vi "Sreen.vi"(1 "IP":string, 2 "Voltage 2":u8, 3 "Voltage 1":u8, 4 "Battery":u8) -> ()   [LabVIEW 2024]
panel:
  out "Port":dbl
  in  "Send":bool
  # "OED Screen Control"
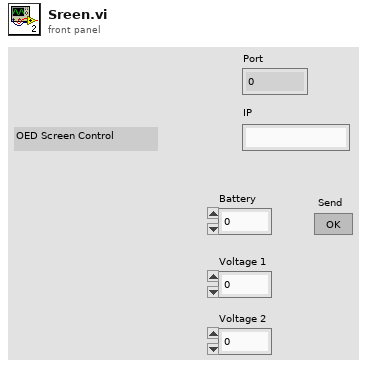
[diagram p1: front panel]
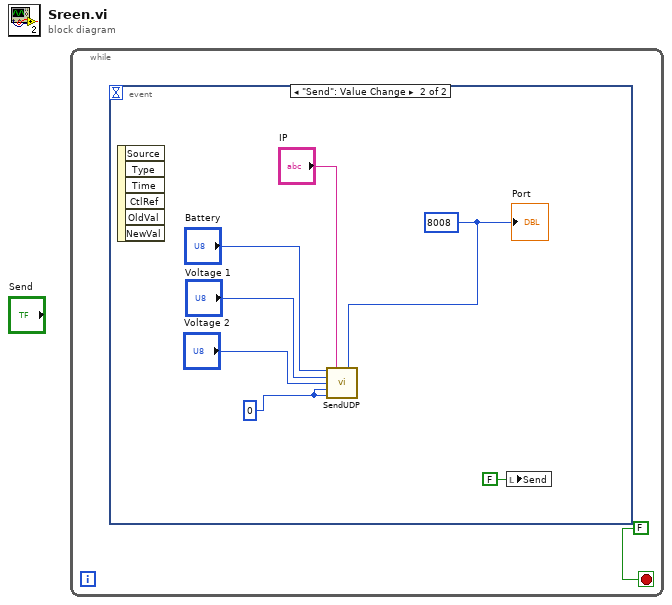
[diagram p0: block diagram]
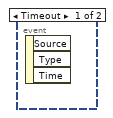
[diagram p2: hidden frame]
diagram:
  n1 = while {
    stop <- FALSE stop-if-true
    n2 = event shown="[1] \"Send\": Value Change" {
      selector: _ -> [_ _]
      dyn-events: _ -> [_ _]
      timeout: _ -> [_ _]
      event Timeout {
        n3 = event-data() -> ()  [unwired: 1 in, 3 out]
      }
      event "Send": Value Change {
        w2 = 0
        w7 = 8008
        n4 = event-data() -> ()  [unwired: 1 in, 6 out]
        n5 = call "SendUDP.vi"("Arg3"="Battery", "IP"="IP", "Port"=w7, "Arg4"="Voltage 1", "Arg5"="Voltage 2", "Arg6"=w2, "Arg7"=w2) -> ()  [unwired: 9 in]
        n6 = local write "Send"(FALSE ("Send")) -> ()
        "Port" <- w7
      }
    }
  }
